vi "Send Alignment Done Event.vi"(8 "error in (no error)":errorcluster caption="에러 입력(에러 없음)", 10 "id":string, 11 "Instrument Manager 입력":refnum<class "Instrument Manager.lvclass">) -> (0 "error out":errorcluster caption="에러 출력", 3 "Instrument Manager 출력":refnum<class "Instrument Manager.lvclass">)   [LabVIEW 2023, in "Instrument Manager.lvclass"]
uses:
  Instrument Manager.lvclass
  Instrument Manager.lvclass/Instrument Manager.ctl
  Error Event.ctl
  Alignment Done Event.ctl
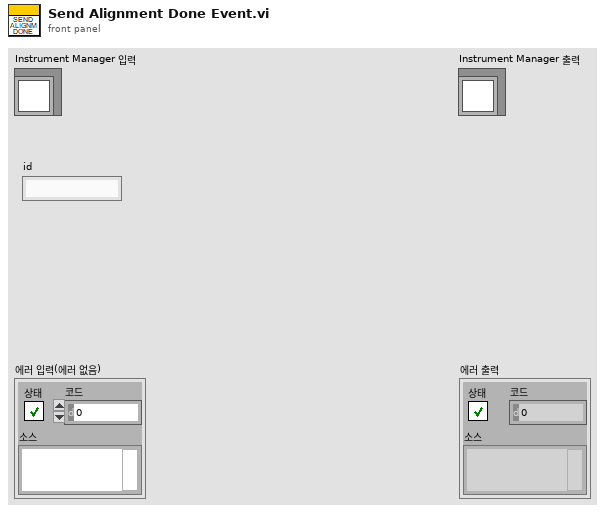
[diagram p1: front panel]
types:
  T1 = typedef "Instrument Manager.lvclass/Alignment Done Event.ctl" = cluster{"type":string, "id":string, "target":string, "command":string}
  T2 = cluster{"Reader Q":refnum<queue>, "Writer Q":refnum<queue>}
  T3 = typedef "Instrument Manager.lvclass/Error Event.ctl" = cluster{"type":string, "id":string, "target":string, "command":string, "Params":cluster{"message ":string}}
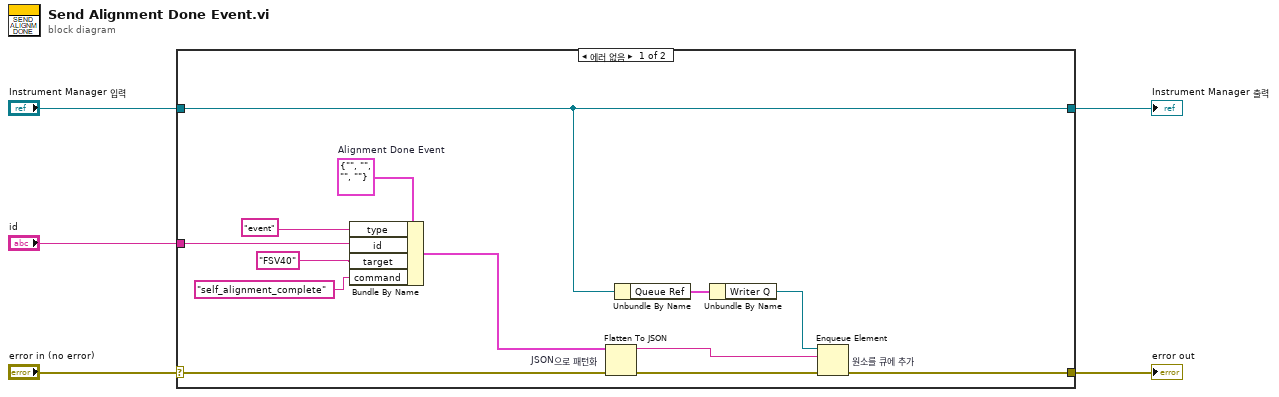
[diagram p0: block diagram]
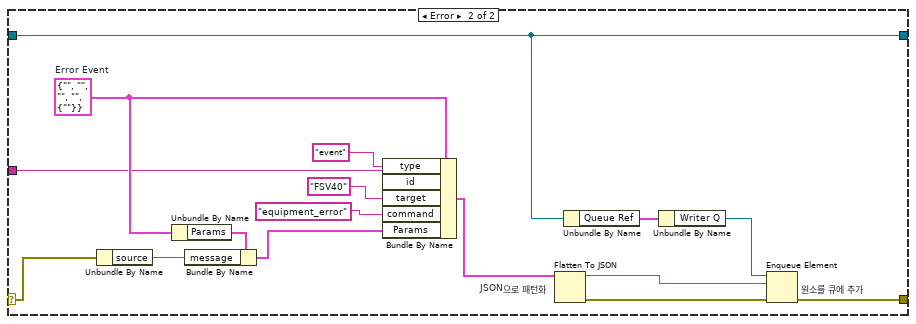
[diagram p2: hidden frame]
diagram:
  n1 = case shown="에러 없음" "error in (no error)" {
    selector: "error in (no error)" -> [w10 w29]
    tunnel: [w8 w30] -> w1
    tunnel: [w7 w20] -> w2
    tunnel: "Instrument Manager 입력" -> [w7 w20]
    tunnel: "id" -> [w14 w24]
    frame No Error {
      w6 = T1 {"type"="", "id"="", "target"="", "command"=""}  # Alignment Done Event
      n2 = Bundle By Name(cluster=w6, "type"="event", "id"=w14, "target"="FSV40", "command"="self_alignment_complete") -> (w11:T1)
      n3 = Flatten To JSON "JSON으로 패턴화"(anything=w11, error in (no error)=w10) -> (JSON string=w16:string, 11:w9:errorcluster)  [unwired: 1 in]
      n4 = Unbundle By Name(w7) -> ("Queue Ref"=w18:T2)
      n5 = Unbundle By Name(w18) -> ("Writer Q"=w17:refnum<queue>)
      n6 = Enqueue Element "원소를 큐에 추가"(queue=w17, element=w16, error in (no error)=w9) -> (error out=w8:errorcluster)  [unwired: 1 in, 2 out]
    }
    frame Error {
      w28 = T3 {"type"="", "id"="", "target"="", "command"="", "Params"={"message "=""}}  # Error Event
      n7 = Unbundle By Name(w29) -> ("source"=w26:string)
      n8 = Unbundle By Name(w28) -> ("Params"=w27:cluster{"message ":string})
      n9 = Bundle By Name(cluster=w27, "message"=w26) -> (w25:cluster{"message ":string})
      n10 = Bundle By Name(cluster=w28, "type"="event", "id"=w24, "target"="FSV40", "command"="equipment_error", "Params"=w25) -> (w19:T3)
      n11 = Flatten To JSON "JSON으로 패턴화"(anything=w19) -> (JSON string=w32:string, 11:w31:errorcluster)  [unwired: 2 in]
      n12 = Unbundle By Name(w20) -> ("Queue Ref"=w34:T2)
      n13 = Unbundle By Name(w34) -> ("Writer Q"=w33:refnum<queue>)
      n14 = Enqueue Element "원소를 큐에 추가"(queue=w33, element=w32, error in (no error)=w31) -> (error out=w30:errorcluster)  [unwired: 1 in, 2 out]
    }
  }
  "error out" <- w1
  "Instrument Manager 출력" <- w2
